vi "all_tests.vi"() -> ()   [LabVIEW 2020]
panel:
  in  "error in":errorcluster
  out "error out":errorcluster
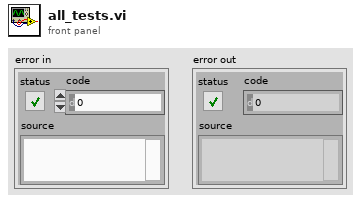
[diagram p1: front panel]
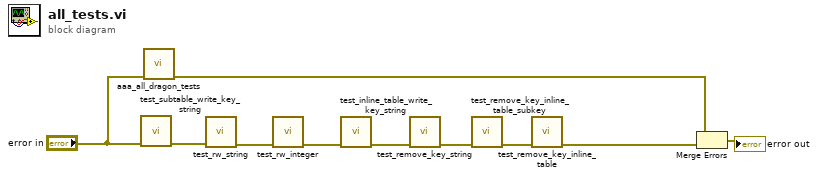
[diagram p0: block diagram]
diagram:
  n1 = call "test_subtable_write_key_string.vi"("error in (no error)"="error in") -> ("error out"=w9:errorcluster)  [unwired: 10 in]
  n2 = call "aaa_all_dragon_tests.vi"("error in (no error)"="error in") -> ("error out"=w5:errorcluster)  [unwired: 10 in]
  n3 = call "test_rw_string.vi"("error in (no error)"=w9) -> ("error out"=w10:errorcluster)  [unwired: 10 in]
  n4 = call "test_rw_integer.vi"("error in (no error)"=w10) -> ("error out"=w8:errorcluster)  [unwired: 10 in]
  n5 = call "test_inline_table_write_key_string.vi"("error in (no error)"=w8) -> ("error out"=w2:errorcluster)  [unwired: 10 in]
  n6 = call "test_remove_key_string.vi"("error in (no error)"=w2) -> ("error out"=w4:errorcluster)  [unwired: 10 in]
  n7 = call "test_remove_key_inline_table_subkey.vi"("error in (no error)"=w4) -> ("error out"=w3:errorcluster)  [unwired: 10 in]
  n8 = call "test_remove_key_inline_table.vi"("error in (no error)"=w3) -> ("error out"=w1:errorcluster)  [unwired: 10 in]
  n9 = Merge Errors(w5, w1) -> (→"error out":errorcluster)
